vi "PicoScope6000GetStreamingValues.vi"(8 "error in":errorcluster, 11 "handle in":i16) -> (0 "error out":errorcluster, 1 "Trigger":cluster{bool, "triggeredAt":u32}, 2 "Start Index":u32, 3 "handle out":i16, 4 "Number of Samples":u32, 5 "ready":i16, 6 "Auto Stopped":bool)   [LabVIEW 2016]
doc: "This VI is used in streaming mode to get the latest values from the driver. It should be called in a loop after the oscilloscope has been set up using PicoScope6000Settings.vi and streaming has been started by calling PicoScope4000StartStreaming.vi. The VI outputs the number of samples available and the start index of these samples in the array output by PicoScope6000StartStreaming.vi."
uses:
  ps6000Wrap.dll
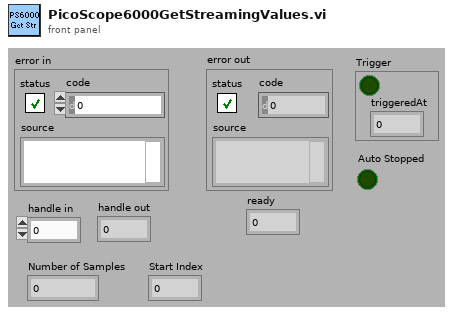
[diagram p1: front panel]
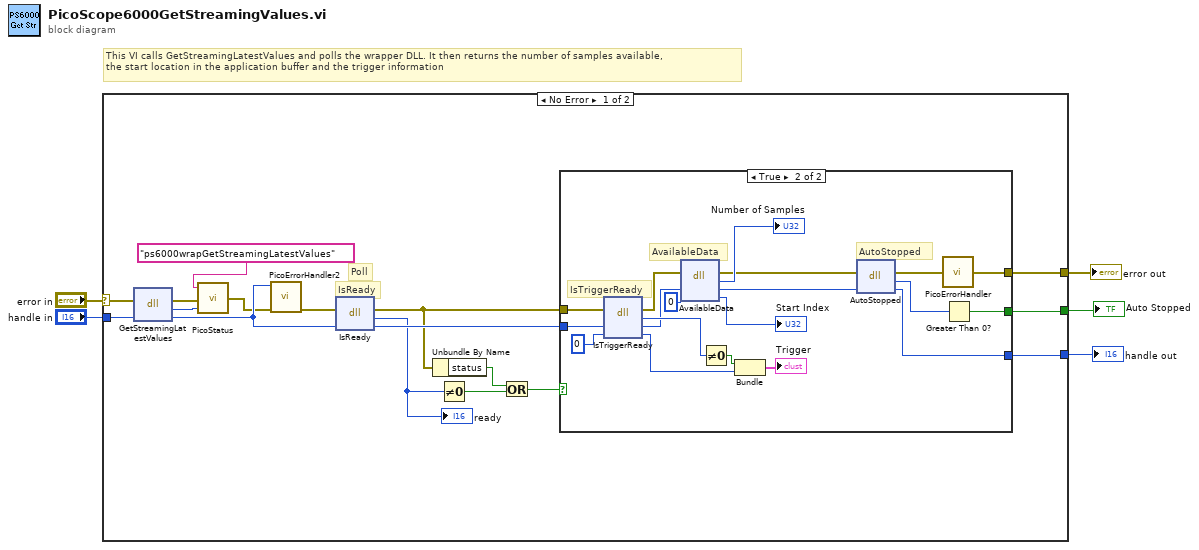
[diagram p0: block diagram]
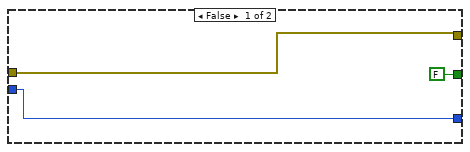
[diagram p2: hidden frame]
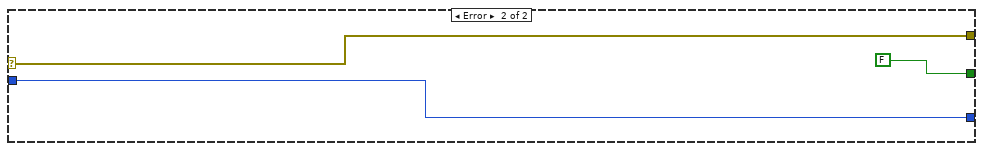
[diagram p3: hidden frame]
diagram:
  # "This VI calls GetStreamingLatestValues and polls the wrapper DLL. It then returns the number of samples available, \nthe start location in the application buffer and the trigger information"
  n1 = case shown="No Error" "error in" {
    selector: "error in" -> [w20 w47]
    tunnel: [w22 w47] -> w4
    tunnel: "handle in" -> [w21 w46]
    tunnel: [w16 w46] -> w2
    tunnel: [w17 FALSE] -> w1
    frame No Error {
      # "Poll"
      # "IsReady"
      n2 = dll-call lib="ps6000wrap.dll" fn="GetStreamingLatestValues" ("PS5000.dll:_ps5000SetDataBuffer@16")(error in=w20, "handle"=w21) -> (error out=w13:errorcluster, "PICO_STATUS"=w12:u32, "handle"=w8:i16)  [unwired: 2 in, 1 out]
      n3 = call "PicoStatus.vi"("PICO STATUS"=w12, "error in"=w13, "source"="ps6000wrapGetStreamingLatestValues") -> ("error out"=w7:errorcluster)
      n4 = call "PicoErrorHandler2.vi"("error in (no error)"=w7, "handle In"=w8) -> ("error out"=w6:errorcluster)  [unwired: 9 in]
      n5 = dll-call lib="ps6000wrap.dll" fn="IsReady" ("PS5000.dll:_ps5000SetDataBuffer@16")(error in=w6, "handle"=w8) -> (error out=w18:errorcluster, "ready"=w14:i16, "handle"=w19:i16)  [unwired: 2 in, 1 out]
      "ready" <- w14
      n6 = Unbundle By Name(w18) -> ("status"=w10:bool)
      n7 = Not Equal To 0?(x=w14) -> (x != 0?=w15:bool)
      n8 = Or(x=w10, y=w15) -> (x .or. y?=w9:bool)
      n9 = case shown="True" w9 {
        tunnel: [w25 w44] -> w22
        tunnel: w19 -> [w24 w42]
        tunnel: w18 -> [w25 w35]
        tunnel: [FALSE w28] -> w17
        tunnel: [w24 w26] -> w16
        frame False {
        }
        frame True {
          # "AutoStopped"
          # "AvailableData"
          # "IsTriggerReady"
          n10 = dll-call lib="ps6000wrap.dll" fn="IsTriggerReady" ("PS5000.dll:_ps5000SetDataBuffer@16")(error in=w35, "handle"=w42, "triggeredAt"=u32 0) -> (error out=w37:errorcluster, "triggered"=w41:i16, "handle"=w36:i16, "triggeredAt"=w39:u32)  [unwired: 2 in, 1 out]
          n11 = dll-call lib="ps6000wrap.dll" fn="AvailableData" ("PS5000.dll:_ps5000Stop@4")(error in=w37, "handle"=w36, "startIndex"=u32 0) -> (error out=w31:errorcluster, "numSamples"=→"Number of Samples":u32, "handle"=w30:i16, "startIndex"=→"Start Index":u32)  [unwired: 2 in, 1 out]
          n12 = Not Equal To 0?(x=w41) -> (x != 0?=w40:bool)
          n13 = Bundle(w40, "triggeredAt"=w39) -> (→"Trigger":cluster{bool, "triggeredAt":u32})  [unwired: 1 in]
          n14 = dll-call lib="ps6000wrap.dll" fn="AutoStopped"(error in=w31, "handle"=w30) -> (error out=w27:errorcluster, "autoStopped"=w29:i16, "handle"=w26:i16)  [unwired: 2 in, 1 out]
          n15 = call "PicoErrorHandler.vi"("error in"=w27) -> ("error out"=w44:errorcluster)
          n16 = Greater Than 0?(x=w29) -> (x > 0?=w28:bool)
        }
      }
    }
    frame Error {
    }
  }
  "error out" <- w4
  "handle out" <- w2
  "Auto Stopped" <- w1
